vi "Izhikevich_Neuron.vi"(0 "I":dbl, 1 "v(t)":dbl, 2 "u(t)":dbl, 3 "dt":dbl, 4 "a":dbl, 5 "Spike Count In":i32, 6 "b":dbl, 8 "c":dbl, 10 "d":dbl) -> (16 "Spike Count Out":i32, 17 "u(t+dt)":dbl, 18 "Spike detected":bool, 19 "v(t+dt)":dbl)   [LabVIEW 2025]
panel:
  # "Outputs:"
  # "Parameters of Izhickevich model :"
  # "Dynamic input:"
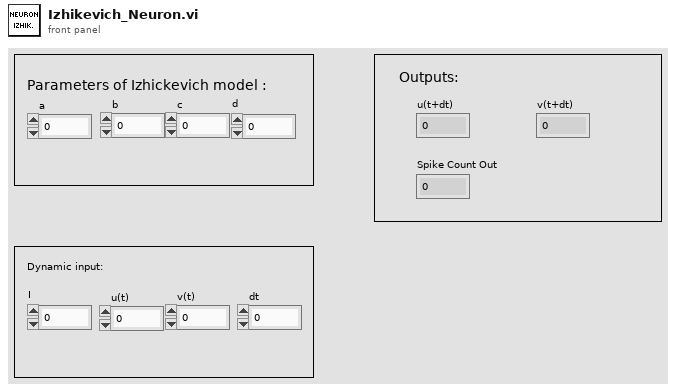
[diagram p1: front panel]
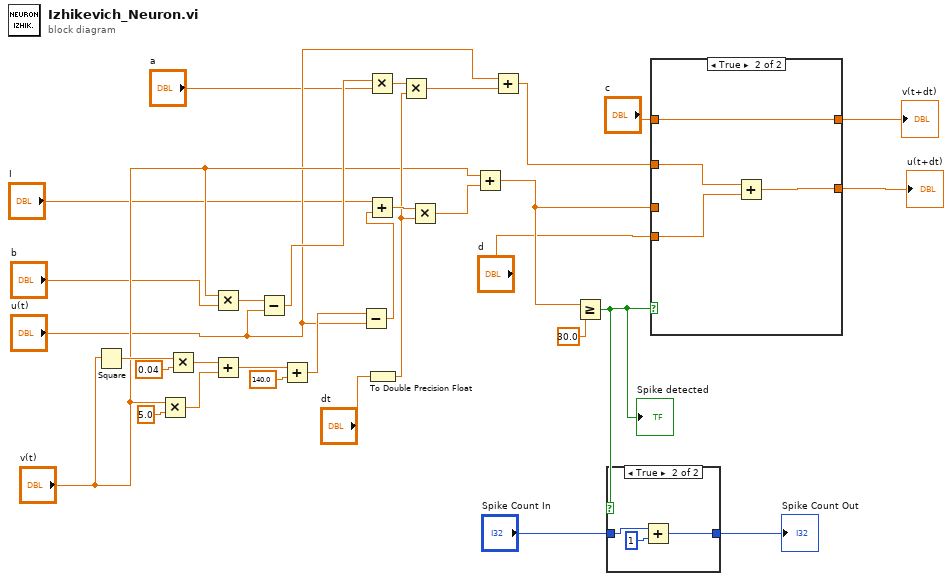
[diagram p0: block diagram]
diagram:
  n1 = Square(x="v(t)") -> (x^2=w32:dbl)
  n2 = Multiply(x="v(t)", y=5.0 ("par 3 giusto")) -> (x*y=w30:dbl)
  n3 = Multiply(x=w32, y=0.04 ("par2 real")) -> (x*y=w31:dbl)
  n4 = Multiply(x="v(t)", y="b") -> (x*y=w24:dbl)
  n5 = Add(x=w31, y=w30) -> (x+y=w29:dbl)
  n6 = Subtract(x=w24, y="u(t)") -> (x-y=w23:dbl)
  n7 = Add(x=w29, y=140.0 ("par 1 giusto")) -> (x+y=w28:dbl)
  n8 = Subtract(x=w28, y="u(t)") -> (x-y=w27:dbl)
  n9 = Multiply(x=w23, y="a") -> (x*y=w3:dbl)
  n10 = Add(x="I", y=w27) -> (x+y=w26:dbl)
  n11 = To Double Precision Float(number="dt") -> (double precision float=w22:dbl)
  n12 = Multiply(x=w3, y=w22) -> (x*y=w21:dbl)
  n13 = Multiply(x=w26, y=w22) -> (x*y=w25:dbl)
  n14 = Add(x="v(t)", y=w25) -> (x+y=w19:dbl)
  n15 = Add(x="u(t)", y=w21) -> (x+y=w18:dbl)
  n16 = Greater Or Equal?(x=w19, y=30.0) -> (x >= y?=w1:bool)
  "Spike detected" <- w1
  n17 = case shown="True" w1 {
    tunnel: "Spike Count In" -> [w33 w35]
    tunnel: [w33 w34] -> w16
    frame False {
    }
    frame True {
      n18 = Add(x=w35, y=1) -> (x+y=w34:i32)
    }
  }
  "Spike Count Out" <- w16
  n19 = case shown="True" w1 {
    tunnel: [w38 w42] -> w5
    tunnel: w19 -> [w38 _]
    tunnel: w18 -> [w37 w39]
    tunnel: [w37 w41] -> w6
    tunnel: "c" -> [_ w42]
    tunnel: "d" -> [_ w40]
    frame False {
    }
    frame True {
      n20 = Add(x=w39, y=w40) -> (x+y=w41:dbl)
    }
  }
  "u(t+dt)" <- w6
  "v(t+dt)" <- w5
